vi "Connect.vi"(8 "error in (no error)":errorcluster, 10 "Connection String":string, 11 "PostgresqlConnection in":refnum<class "DBC.lvclass">) -> (0 "error out":errorcluster, 3 "PostgresqlConnection out":refnum<class "DBC.lvclass">)   [LabVIEW 2020, in "ORM_sqlite_jdp.lvlib" / "DBC.lvclass"]
uses:
  DBC.lvclass
  C:/Program Files/National Instruments/LabVIEW 2020/vi.lib/Viviota/shared/ORM.lvlibp/DbConnection/DbConnection.lvclass
  <vilib>/drjdpowell/SQLite Library/SQL Connection/Connection.lvclass
  DBC.lvclass/DBC.ctl
  <vilib>/drjdpowell/SQLite Library/SQL Connection/Open (string).vi
  Write Connection.vi
  <vilib>/Viviota/shared/ORM.lvlibp/DbConnection/Write ColumnNameEqualsValueFormat.vi
  <vilib>/Viviota/shared/ORM.lvlibp/DbConnection/Write ColumnNameFormat.vi
  <vilib>/Viviota/shared/ORM.lvlibp/DbConnection/Write LastIdentityQuery.vi
  <vilib>/Viviota/shared/ORM.lvlibp/DbConnection/Write TableNameFormat.vi
  <vilib>/regexp/Match Regular Expression.xnode
panel:
  # "host = hostname\nhostaddr = ipaddress\nport\ndbname\nuser\npassword\nsslmode\nrequiressl (0 or 1)\nconnect_timeout"
  # "host=localhost port=5432 dbname = mydb"
  # "https://www.postgresql.org/docs/17/libpq-connect.html#LIBPQ-PARAMKEYWORDS"
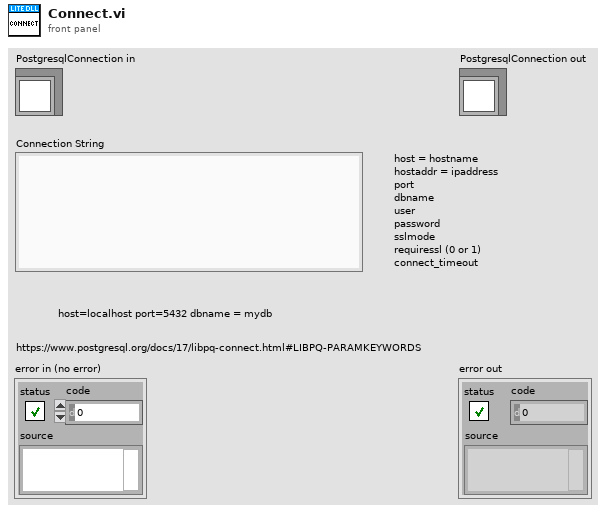
[diagram p1: front panel]
types:
  T1 = enum16{"New or existing", "Existing", "Read only"}
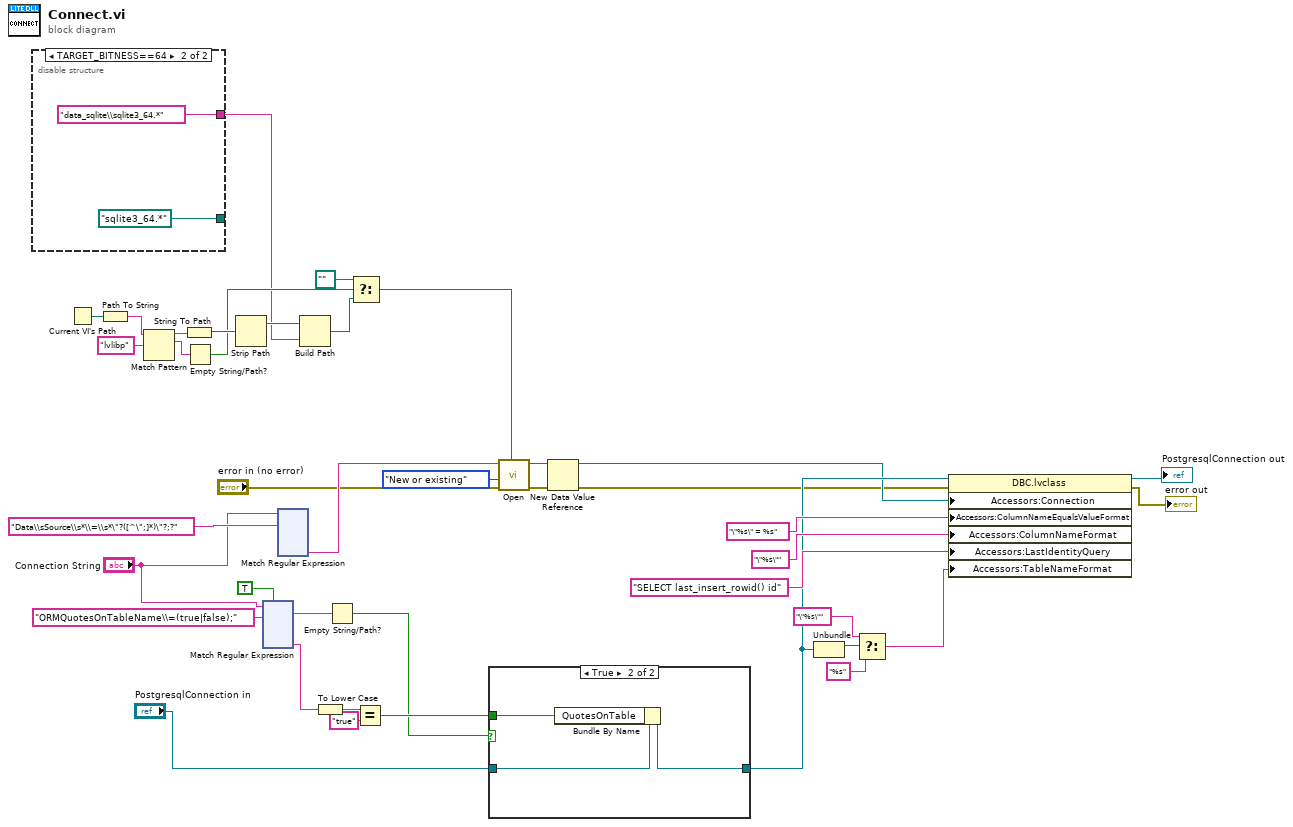
[diagram p0: block diagram]
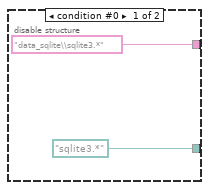
[diagram p2: hidden frame]
diagram:
  n1 = disable-structure shown="TARGET_BITNESS==64" {
    disable-tunnel: ["data_sqlite\\sqlite3.*" ("name or relative path") "data_sqlite\\sqlite3_64.*" ("name or relative path")] -> w3
    disable-tunnel: [path "sqlite3.*" ("Application Directory") path "sqlite3_64.*" ("Application Directory")] -> _
    frame condition #0 {
    }
    frame condition #1 (active) {
    }
  }
  n2 = Current VI's Path() -> (path=w13:path)
  n3 = Path To String(path=w13) -> (string=w12:string)
  n4 = Match Pattern(string=w12, regular expression="lvlibp") -> (before substring=w10:string, match substring=w9:string)  [unwired: 1 in, 2 out]
  n5 = String To Path(string=w10) -> (path=w8:path)
  n6 = Empty String/Path?(string/path=w9) -> (empty?=w6:bool)
  n7 = Strip Path(path=w8) -> (stripped path=w7:path)  [unwired: 1 out]
  n8 = xnode "Match Regular Expression"("input string"="Connection String", "regular expression"="ORMQuotesOnTableName\\=(true|false);", "ignore case? (F)"=TRUE) -> ("whole match"=w32:string, "submatch 1"=w31:string)  [unwired: 3 in, 4 out]
  n9 = xnode "Match Regular Expression"("input string"="Connection String", "regular expression"="Data\\sSource\\s*\\=\\s*\"?([^\";]*)\"?;?") -> ("submatch 1"=w20:string)  [unwired: 4 in, 5 out]
  n10 = Build Path(base path=w7, name or relative path=w3) -> (appended path=w5:path)
  n11 = To Lower Case(string=w31) -> (all lower case string=w30:string)
  n12 = Empty String/Path?(string/path=w32) -> (empty?=w27:bool)
  n13 = Select(t=path "", s=w6, f=w5) -> (s? t:f=w2:path)
  n14 = Equal?(x=w30, y="true") -> (x = y?=w28:bool)
  n15 = case shown="True" w27 {
    tunnel: "PostgresqlConnection in" -> [w45 w48]
    tunnel: [w45 w47] -> w25
    tunnel: w28 -> [_ w46]
    frame False {
    }
    frame True {
      n16 = Bundle By Name(cluster=w48, "QuotesOnTable"=w46) -> (w47:refnum<class "DBC.lvclass">)
    }
  }
  n17 = call-poly <vilib>:"Open.vi"("SQLite Library Path"=w2, "error in (no error)"="error in (no error)", "File Option"=T1."New or existing", "db file"=w20) -> ("error out"=w19:errorcluster, "SQLite Connection"=w18:refnum<class "Connection.lvclass">)  [unwired: 6 in]
  n18 = New Data Value Reference(data value=w18, error in=w19) -> (data value reference=w16:refnum<data-value>, error out=w14:errorcluster)
  n19 = Unbundle(w25) -> (w15:bool)  [unwired: 1 out]
  n20 = Select(t="\"%s\"" ("TableNameFormat"), s=w15, f="%s" ("TableNameFormat")) -> (s? t:f=w35:string)
  n21 = property class="DBC.lvclass"(reference=w25, error in=w14, "Accessors:Connection"=w16, "Accessors:ColumnNameEqualsValueFormat"="\"%s\" = %s" ("ColumnNameFormat"), "Accessors:ColumnNameFormat"="\"%s\"" ("ColumnNameFormat"), "Accessors:LastIdentityQuery"="SELECT last_insert_rowid() id" ("LastIdentityQuery"), "Accessors:TableNameFormat"=w35) -> (reference out=→"PostgresqlConnection out":refnum<class "DBC.lvclass">, error out=→"error out":errorcluster)
